vi "Volume ROI entry user dialogue handler.vi"(7 "Center around clicked pixel (F)":bool, 8 "error in (no error)":errorcluster, 11 "New coordinates":i32[](array[numeric])) -> (0 "error IO":errorcluster, 1 "Cancelled":bool, 3 "ROIs Info []":T1[](array[typedef]) {"FOV" min=1.0 max=10.0 step=1.0; "Frame Size" min=1.0 max=10.0 step=1.0; "Laser Power" min=1.0 max=10.0 step=0.10000000149011612; "Rel. Resolution" min=1.0 max=10.0 step=1.0; "POI Dwell time" min=1.0 max=10.0 step=0.10000000149011612; "Zoom" min=1.0 max=10.0 step=0.10000000149011612})   [LabVIEW 2020]
uses:
  Typedefs/ROI spec.ctl
  Typedefs/ROI ID Enum.ctl
  ROI Entry screen/Globals/gl_ROI Entry UI globals.vi
panel:
  out "Modified coordinates":i32[](array[numeric])
  # "Tick the box below if you want to specify a volume from the rectangular shaped you have drawn and enter select the two z--planes between which the volume should be created."
  # "X1\nY1\nX2\nY2"
  # "X1\nY1\nX2\nY2"
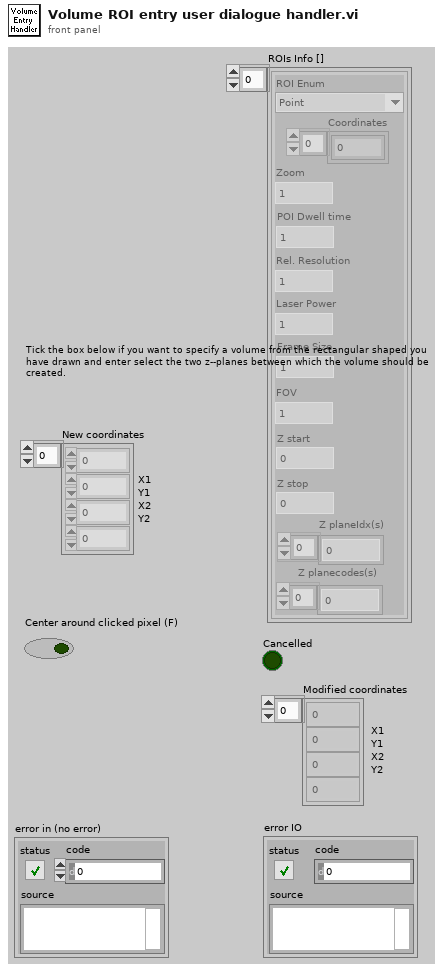
[diagram p1: front panel]
types:
  T1 = typedef "ROI spec.ctl" = cluster{"ROI Enum":T2, "Coordinates":i32[], "Zoom":dbl, "POI Dwell time":dbl, "Rel. Resolution":dbl, "Laser Power":dbl, "Frame Size":dbl, "FOV":dbl, "Z start":dbl, "Z stop":dbl, "Z planeIdx(s)":i32[], "Z planecodes(s)":u8[]}
  T2 = typedef "ROI ID Enum.ctl" = enum16{"Point", "MiniScan", "Comp. MiniScan", "Rectangle", "Comp. volume", "Arb. plane point", "None"}
  T3 = typedef "ROI entry screen ctrl refs cluster.ctl" = cluster{"Done button":refnum<vi>, "Imaging button":refnum<vi>, "Acquisition button":refnum<vi>, "Scan dwell time per pixel (us)":refnum<vi>, "# of planes":refnum<vi>, "Zoom Ctrl":refnum<vi>, "Equal size":refnum<vi>, "Channel":refnum<vi>, "Image Display":refnum<vi>, "Z-Plane Selector":refnum<vi>, "Number of lines left":refnum<vi>, "Z-stack folder path":refnum<vi>, "POI Density":refnum<vi>, "Arb Plane Entry":refnum<vi>, "Whole Plane":refnum<vi>, "Line Mode":refnum<vi>, "Clear Last":refnum<vi>, "Clear All":refnum<vi>, "Delete Lines":refnum<vi>, "Trial Length (sec)":refnum<vi>, "Palette Type":refnum<vi>, "Intensity slider":refnum<vi>, "# POI":refnum<vi>, "Max Z Proj":refnum<vi>, "Zplane ind":refnum<vi>, "Wavelength (nm)":refnum<vi>, "Number of Trials":refnum<vi>, "Funct stim.trig.enable":refnum<vi>, "Funct stim.trig.delay (s)":refnum<vi>, "Line Mode":refnum<vi>, "Step size (µm)":refnum<vi>, "ROI move mode":refnum<vi>, "Cool-down time (s)":refnum<vi>, "Enable cool-down time":refnum<vi>, "Motor Z ind. (um)":refnum<vi>, "AOL Z ind. (um)":refnum<vi>, "Load Reference Image":refnum<vi>, "Rel.  Res.":refnum<vi>, "ROI LIST":refnum<vi>, "Show All":refnum<vi>, "ROI Type":refnum<vi>, "Start Plane":refnum<vi>, "Stop Plane":refnum<vi>, "Offset ROI":refnum<vi>, "Tab Control":refnum<vi>, "Laser Power(%)":refnum<vi>, "Cycle rate":refnum<vi>, "FOV (Ind.)":refnum<vi>, "Frame Size (Ind.)":refnum<vi>, "Resolution (Ind.)":refnum<vi>, "Pixel Density (Ind)":refnum<vi>, "Laser Power (Ind.)":refnum<vi>, "Dwell Time (Ind.)":refnum<vi>, "Adj MC":refnum<vi>}
  T4 = typedef "ROI Z-stack settings info.ctl" = cluster{"Zoom":dbl, "POI Dwell time":dbl, "Rel. Res":dbl, "Laser Power %":dbl, "Frame Size":dbl, "FOV":dbl}
  T5 = typedef "ROI input mode.ctl" = enum16{"Unspecified", "Point-Line-Plane", "Volume"}
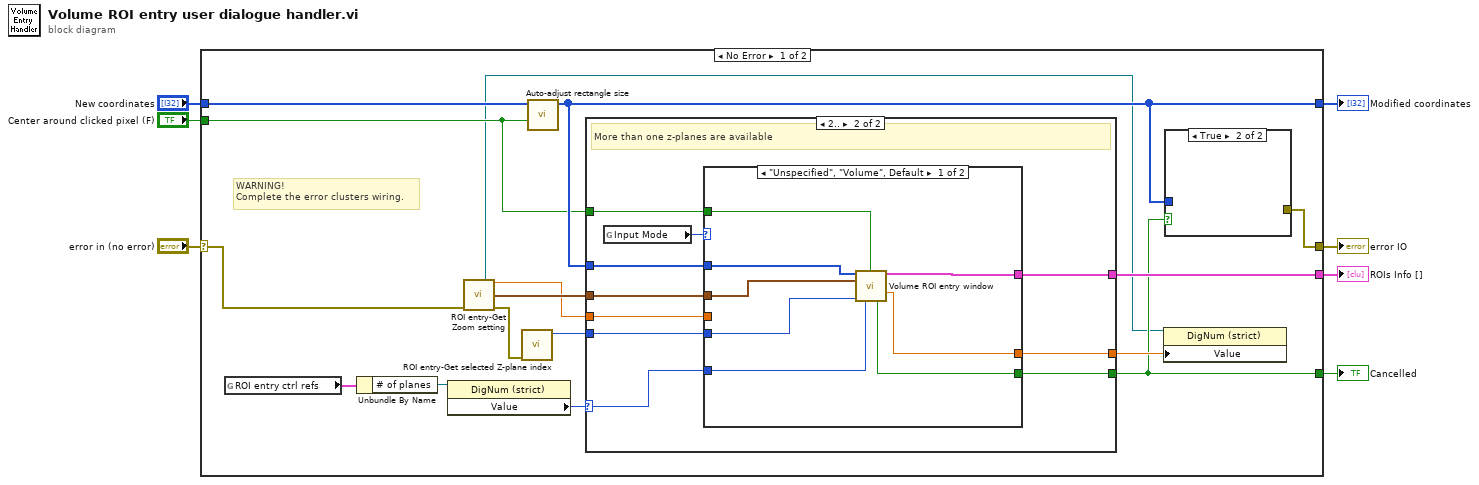
[diagram p0: block diagram]
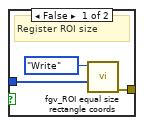
[diagram p2: hidden frame]
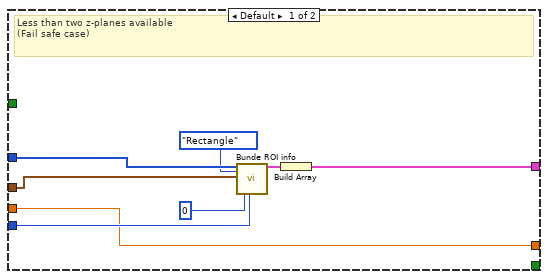
[diagram p3: hidden frame]
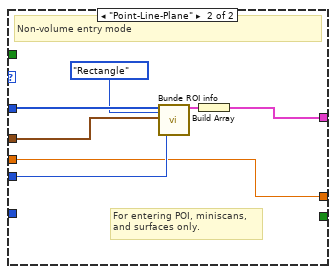
[diagram p4: hidden frame]
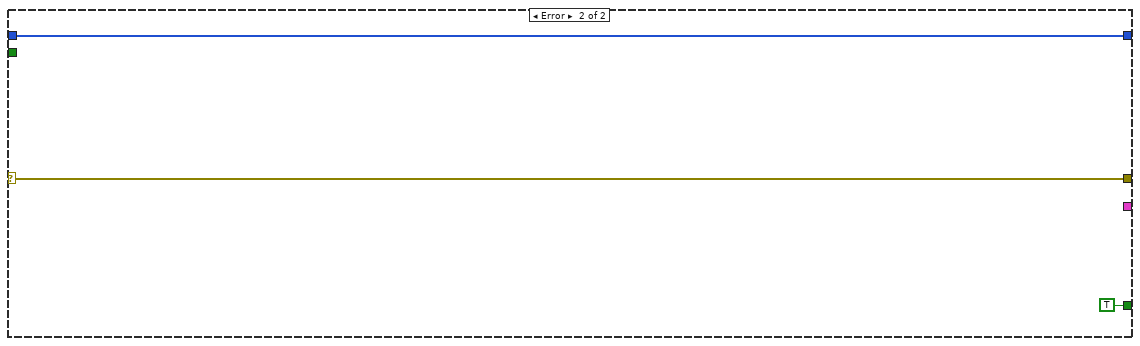
[diagram p5: hidden frame]
diagram:
  n1 = case shown="No Error" "error in (no error)" {
    selector: "error in (no error)" -> [w12 w62]
    tunnel: [w23 _] -> w7
    tunnel: "New coordinates" -> [w22 w60]
    tunnel: [w16 w60] -> w5
    tunnel: [w15 TRUE ("Cancelled")] -> w4
    tunnel: [w13 w62] -> w2
    tunnel: "Center around clicked pixel (F)" -> [w11 _]
    frame No Error {
      # "WARNING!\nComplete the error clusters wiring."
      n2 = global read "gl_ROI Entry UI globals.vi" "ROI entry ctrl refs"() -> (w20:T3)
      n3 = Unbundle By Name(w20) -> ("# of planes"=w21:refnum<vi>)
      n4 = property class="DigNum (strict)"(reference=w21) -> ("Value"=w19:i32)  [unwired: 1 in, 2 out]
      n5 = call "ROI entry-Get Zoom setting.vi"("error in (no error)"=w12) -> ("Zoom control ref"=w10:refnum<vi>, "Zoom Value"=w8:dbl, "AOLZ Settings"=w9:T4, "error out"=w14:errorcluster)  [unwired: 6 in, 5 out]
      n6 = call "ROI entry-Get selected Z-plane index.vi"("error in (no error)"=w14) -> ("Z-plane selector (index)"=w17:i32)  [unwired: 9 in, 1 out]
      n7 = call "Auto-adjust rectangle size.vi"("Center around clicked pixel (F)"=w11, "New Coordinates"=w22) -> ("Modified coordinates"=w16:i32[])  [unwired: 9 in]
      n8 = case shown="2.." w19 {
        selector: w19 -> [_ w41]
        tunnel: [w34 w42] -> w23
        tunnel: w16 -> [w33 w44]
        tunnel: w17 -> [w30 w43]
        tunnel: [_ w40] -> w15
        tunnel: [w27 w38] -> w18
        tunnel: w11 -> [_ w37]
        tunnel: w9 -> [w28 w36]
        tunnel: w8 -> [w27 w35]
        frame Default {
          # "Less than two z-planes available\n(Fail safe case)"
          n9 = call "Bunde ROI info.vi"("ROI Coordinates"=w33, "ROI Enum"=ROI_ID_Enum."Rectangle", "Z stack Settings"=w28, "ZplaneIndex"=u8 0 ("Zplanecode"), "Zplanecode"=w30) -> ("ROI Info"=w32:T1)  [unwired: 14 in]
          n10 = Build Array(w32) -> (w34:T1[])
        }
        frame 2.. {
          # "More than one z-planes are available"
          n11 = global read "gl_ROI Entry UI globals.vi" "Input Mode"() -> (w39:T5)
          n12 = case shown="\"Unspecified\", \"Volume\", Default" w39 {
            tunnel: w44 -> [w52 w58]
            tunnel: w43 -> [w51 w55]
            tunnel: [w50 w59] -> w42
            tunnel: w41 -> [w49 _]
            tunnel: [w48 _] -> w40
            tunnel: [w47 w53] -> w38
            tunnel: w37 -> [w46 _]
            tunnel: w36 -> [w45 w54]
            tunnel: w35 -> [_ w53]
            frame "Unspecified", "Volume", Default {
              n13 = call "Volume ROI entry window.vi"("Coordinates"=w52, "Do not initialise selector values"=w46, "AOLZ Settings"=w45, "ZplaneIndex (zero based)"=w51, "# of planes"=w49) -> ("ROIs Info []"=w50:T1[], "Zoom (out)"=w47:dbl, "Cancelled"=w48:bool)  [unwired: 8 in]
            }
            frame "Point-Line-Plane" {
              # "For entering POI, miniscans,\nand surfaces only."
              # "Non-volume entry mode"
              n14 = call "Bunde ROI info.vi"("ROI Coordinates"=w58, "ROI Enum"=ROI_ID_Enum."Rectangle", "Z stack Settings"=w54, "ZplaneIndex"=w55) -> ("ROI Info"=w57:T1)  [unwired: 15 in]
              n15 = Build Array(w57) -> (w59:T1[])
            }
          }
        }
      }
      n16 = property class="DigNum (strict)"(reference=w10, "Value"=w18) -> ()  [unwired: 1 in, 2 out]
      n17 = case shown="True" w15 {
        tunnel: w16 -> [w26 _]
        tunnel: [w24 _] -> w13
        frame False {
          # "Register ROI size"
          n18 = call "fgv_ROI equal size rectangle coords.vi"("New Rectangle Coordinates"=w26, "Function"=enum16{"Intialize", "Write", "Read", "Clear"}."Write") -> ("error out"=w24:errorcluster)  [unwired: 8 in, 1 out]
        }
        frame True {
        }
      }
    }
    frame Error {
    }
  }
  "ROIs Info []" <- w7
  "Cancelled" <- w4
  "Modified coordinates" <- w5
  "error IO" <- w2
